vi "Write CE BT Power Setting.vi"(8 "error in (no error)":errorcluster, 10 "CE BT Power Setting":T1={"Center and Span Frequency(Hz)"={"Center"=0.0, "Span"=0.0}, "Ref and Atten"={"Reference Level"=0.0, "Atten"=0, "Atten Auto?"=FALSE}, "External Loss"=0.0, "RBW/VBW(Hz)"={"RBW"=0.0, "VBW"=0.0}, "Sweep Point"=0, "Sweep Time(s)"={"Time"=0.0, "Auto?"=FALSE}, "Trace and Detect"=[], "Avg/Hold Number"=0, "Average Mode"=enum."Exponential", "Gate Setting"={"Sweep Time(sec)"=0.0, "Delay(sec)"=0.0, "Length"=0.0, "Source"=enum."RF Burst", "Trigger Level"=0.0}} {"Center and Span Frequency(Hz)"."Span" format="%#_6p"; "Center and Span Frequency(Hz)"."Center" format="%#_6p"; "Sweep Time(s)"."Time" format="%#_6p"; "RBW/VBW(Hz)"."VBW" format="%#_6p"; "RBW/VBW(Hz)"."RBW" format="%#_6p"}, 11 "SA Measurement in":refnum<class "SA Measurement.lvclass">) -> (0 "error out":errorcluster, 3 "SA Measurement out":refnum<class "SA Measurement.lvclass">)   [LabVIEW 2023, in "Spectrum Analyzer.lvlib" / "SA Measurement.lvclass"]
uses:
  SA Measurement.lvclass
  TYPE DEFINITION/SA Measurement Class/TYPE CE BT Power Setting Parameter.ctl
  TYPE DEFINITION/TYPE Center and Span Frequency.ctl
  TYPE DEFINITION/TYPE Reference Level and Atten Param.ctl
  TYPE DEFINITION/TYPE Display Trace Mode Select.ctl
  TYPE DEFINITION/TYPE Detect Mode Select.ctl
  SA Measurement.lvclass/SA Measurement.ctl
  Spectrum Analyzer.lvlib
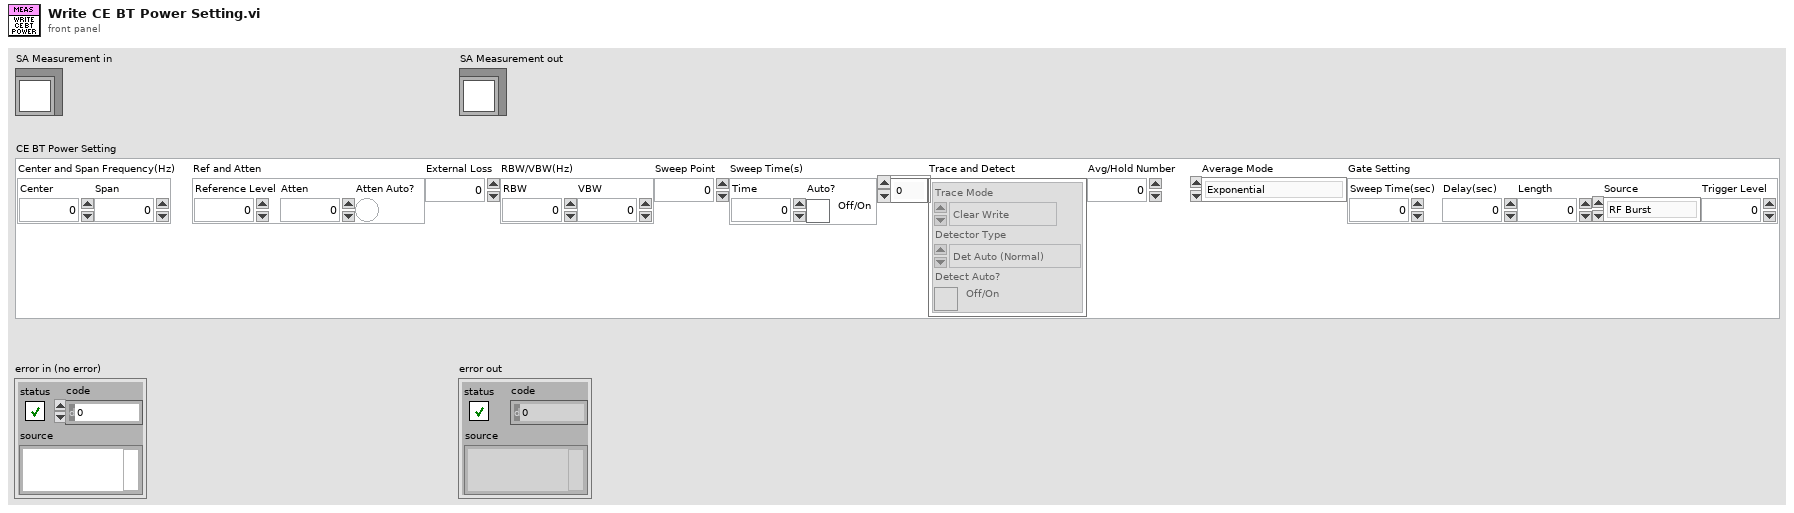
[diagram p1: front panel]
types:
  T1 = typedef "Spectrum Analyzer.lvlib/TYPE CE BT Power Setting Parameter.ctl" = cluster{"Center and Span Frequency(Hz)":T2, "Ref and Atten":T3, "External Loss":dbl, "RBW/VBW(Hz)":cluster{"RBW":dbl, "VBW":dbl}, "Sweep Point":u32, "Sweep Time(s)":cluster{"Time":dbl, "Auto?":bool}, "Trace and Detect":cluster{"Trace Mode":T4, "Detector Type":T5, "Detect Auto?":bool}[], "Avg/Hold Number":u32, "Average Mode":enum16{"Exponential", "Repeat"}, "Gate Setting":cluster{"Sweep Time(sec)":dbl, "Delay(sec)":dbl, "Length":dbl, "Source":enum16{"External 1", "External 2", "Line", "Frame", "RF Burst", "TV", "PXI"}, "Trigger Level":dbl}}
  T2 = typedef "Spectrum Analyzer.lvlib/TYPE Center and Span Frequency.ctl" = cluster{"Center":dbl, "Span":dbl}
  T3 = typedef "Spectrum Analyzer.lvlib/TYPE Reference Level and Atten Param.ctl" = cluster{"Reference Level":dbl, "Atten":i32, "Atten Auto?":bool}
  T4 = typedef "Spectrum Analyzer.lvlib/TYPE Display Trace Mode Select.ctl" = enum16{"Clear Write", "Max Hold", "Min Hold", "Average", "View"}
  T5 = typedef "Spectrum Analyzer.lvlib/TYPE Detect Mode Select.ctl" = enum16{"Det Auto (Normal)", "Auto Peak", "Positive Peak", "Negative Peak", "Sample", "RMS", "Average", "Quasipeak", "CISPR Average", "RMS Average"}
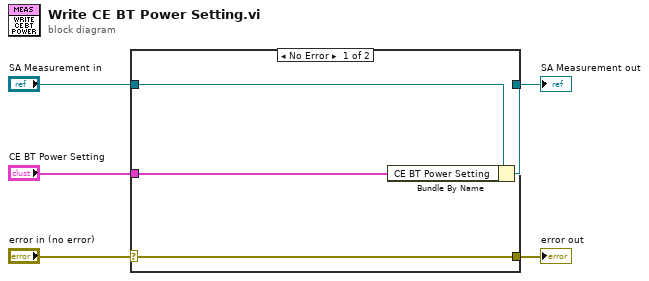
[diagram p0: block diagram]
diagram:
  n1 = case shown="No Error" "error in (no error)" {
    selector: "error in (no error)" -> [w9 w10]
    tunnel: [w9 w10] -> w4
    tunnel: [w7 w11] -> w2
    tunnel: "SA Measurement in" -> [w8 w11]
    tunnel: "CE BT Power Setting" -> [w6 _]
    frame No Error {
      n2 = Bundle By Name(cluster=w8, "CE BT Power Setting"=w6) -> (w7:refnum<class "SA Measurement.lvclass">)
    }
    frame Error {
    }
  }
  "error out" <- w4
  "SA Measurement out" <- w2
